vi "Measurement UI.vi"() -> ()   [LabVIEW 2024, in "NIDmmDcRmsMeasurement.lvlib"]
uses:
  NIDmmDCRmsMeasurement.lvlib
panel:
  out "Waveform Data":dbl[](array[numeric]) caption="Waveform Waveform"
  out "Measurement Waveform":waveform(dbl)(graph)
  out "RMS Value":dbl
  out "DC Value":dbl
  out "Signal Out of Range":bool
  in  "Sample Rate (Hz)":dbl=1800000.0 caption="Pin Name" format="%.2p"
  in  "Number of Samples":i32=1000 caption="Sample Rate (Hz)"
  in  "Function":i32(ring)=1003 caption="Measurement Type" items=["Waveform Voltage"=1003, "Waveform Current"=1004]
  in  "Range":dbl=10.0
  in  "Pin Name":string(combo)="Pin1"
  # "Input"
  # "Output"
  # "Pin Settings"
  # "Timing Settings"
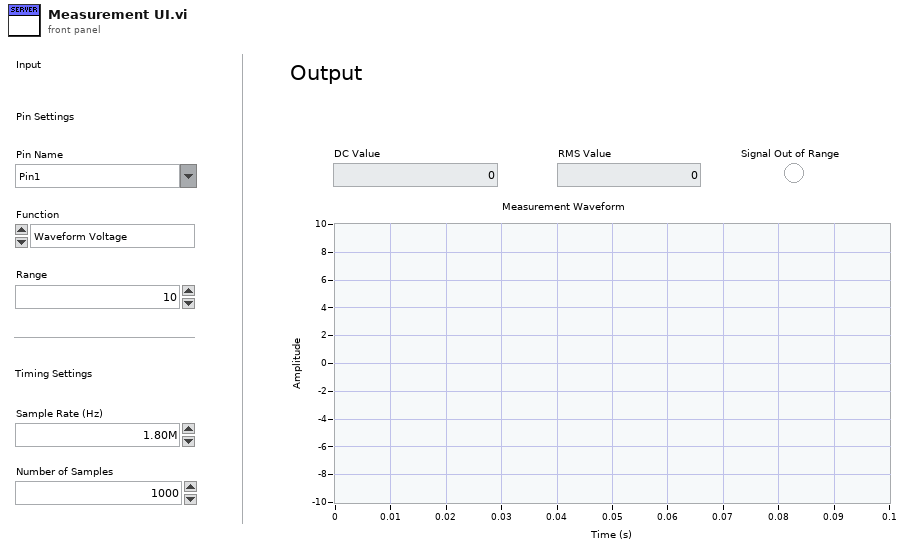
[diagram p1: front panel]
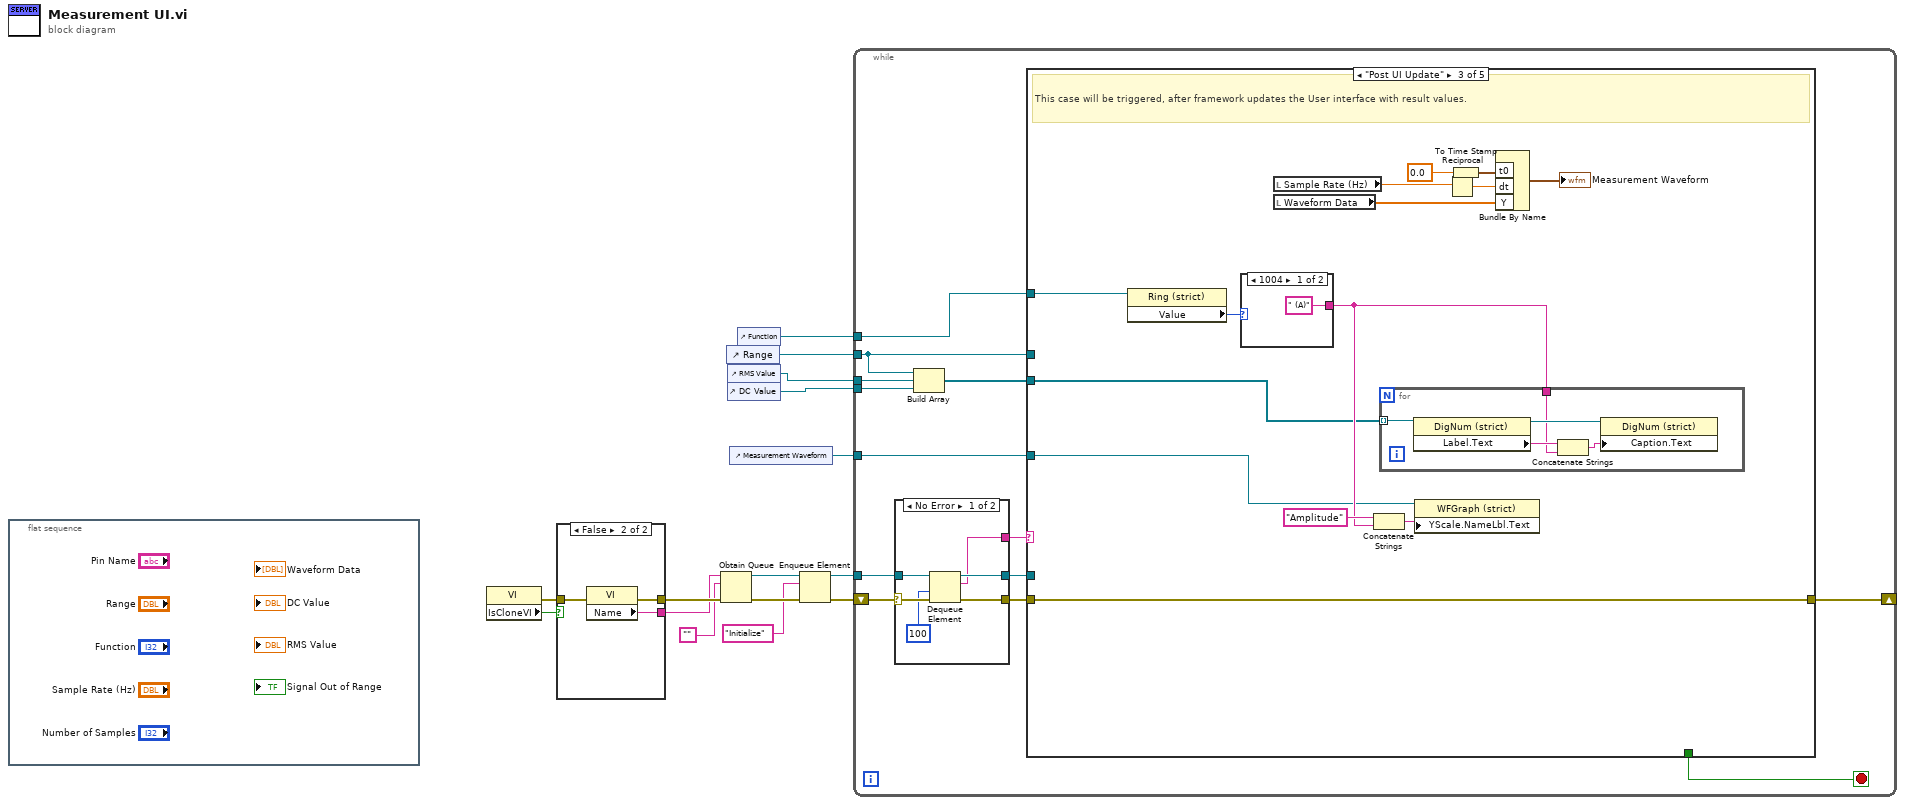
[diagram p0: block diagram]
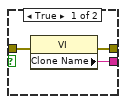
[diagram p2: hidden frame]
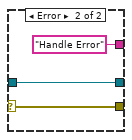
[diagram p3: hidden frame]
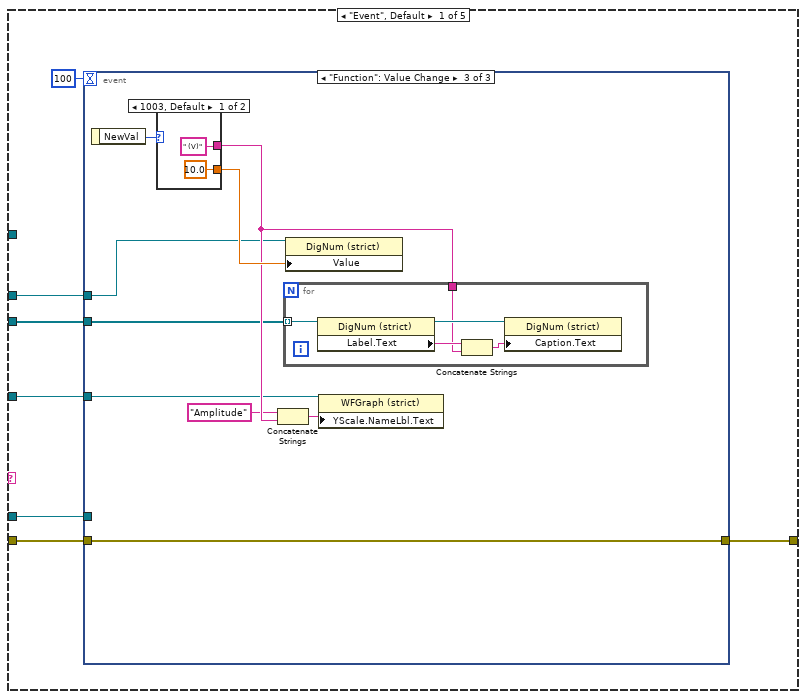
[diagram p4: hidden frame]
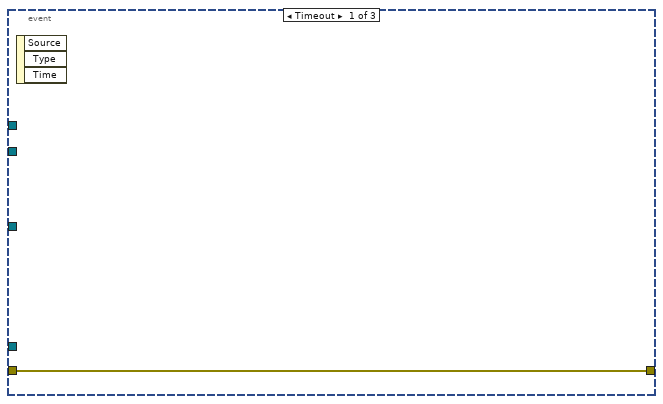
[diagram p5: hidden frame]
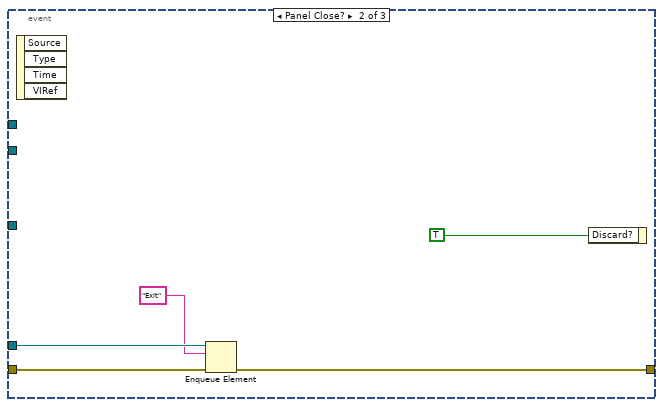
[diagram p6: hidden frame]
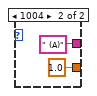
[diagram p7: hidden frame]
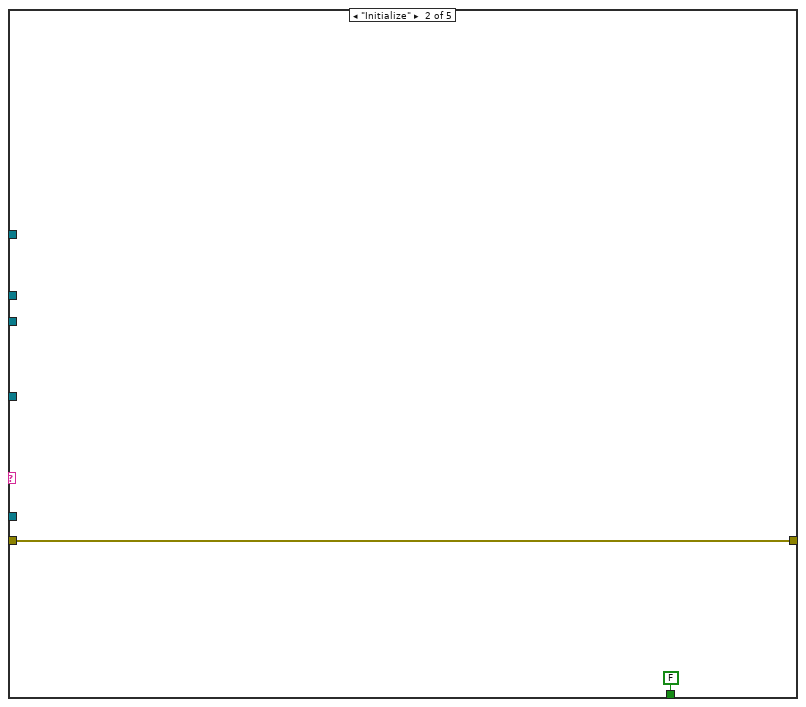
[diagram p8: hidden frame]
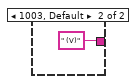
[diagram p9: hidden frame]
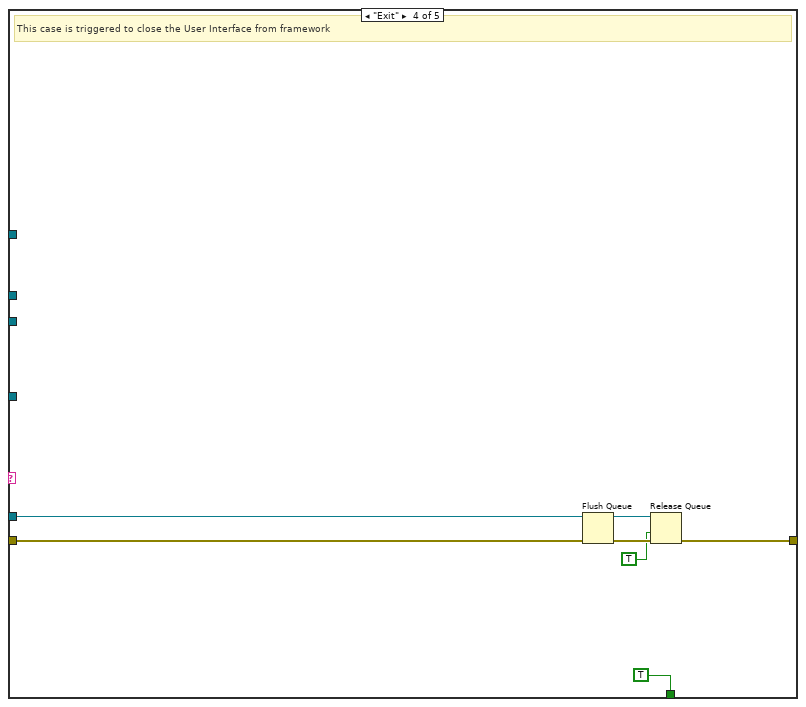
[diagram p10: hidden frame]
diagram:
  n1 = flat-sequence {
    frame #0 {
    }
  }
  n2 = property class="VI"() -> (error out=w6:errorcluster, "IsCloneVI"=w7:bool)  [unwired: 2 in, 1 out]
  n3 = case shown="False" w7 {
    tunnel: [w18 w21] -> w15
    tunnel: [w17 w20] -> w14
    tunnel: w6 -> [w16 w19]
    frame True {
      n4 = property class="VI"(error in=w16) -> (error out=w18:errorcluster, "Clone Name"=w17:string)  [unwired: 1 in, 1 out]
    }
    frame False {
      n5 = property class="VI"(error in=w19) -> (error out=w21:errorcluster, "Name"=w20:string)  [unwired: 1 in, 1 out]
    }
  }
  n6 = Obtain Queue(name (unnamed)=w14, element data type="", error in (no error)=w15) -> (queue out=w11:refnum<queue>, error out=w13:errorcluster)  [unwired: 2 in, 1 out]
  n7 = control-ref of="Range"() -> (w4:refnum<vi>)
  n8 = control-ref of="RMS Value"() -> (w3:refnum<vi>)
  n9 = control-ref of="DC Value"() -> (w2:refnum<vi>)
  n10 = control-ref of="Measurement Waveform"() -> (w5:refnum<vi>)
  n11 = control-ref of="Function"() -> (w1:refnum<vi>)
  n12 = Enqueue Element(queue=w11, element="Initialize", error in (no error)=w13) -> (queue out=w10:refnum<queue>, error out=w12:errorcluster)  [unwired: 1 in, 1 out]
  n13 = while {
    shift-right: [w29] -> _
    shift-left: w12 -> [w34]
    tunnel: w10 -> [w32]
    tunnel: w5 -> [w27]
    tunnel: w4 -> [w26]
    tunnel: w3 -> [w24]
    tunnel: w2 -> [w23]
    tunnel: w1 -> [w25]
    stop <- w28 stop-if-true
    n14 = case shown="No Error" w34 {
      selector: w34 -> [w40 w43]
      tunnel: [w39 w43] -> w33
      tunnel: w32 -> [w38 w42]
      tunnel: [w37 w42] -> w31
      tunnel: [w36 "Handle Error"] -> w30
      frame No Error {
        n15 = Dequeue Element(queue=w38, timeout in ms (-1)=100, error in (no error)=w40) -> (queue out=w37:refnum<queue>, element=w36:string, error out=w39:errorcluster)  [unwired: 1 out]
      }
      frame Error {
      }
    }
    n16 = Build Array(w26, w24, w23) -> (w22:refnum<vi>[])
    n17 = case shown="\"Post UI Update\"" w30 {
      tunnel: w33 -> [w49 w76 w90 w104 w105]
      tunnel: w31 -> [w47 _ _ w102 _]
      tunnel: [w50 w76 w90 w99 w105] -> w29
      tunnel: [_ FALSE _ TRUE _] -> w28
      tunnel: w27 -> [w46 _ w77 _ _]
      tunnel: w26 -> [w45 _ _ _ _]
      tunnel: w25 -> [_ _ w79 _ _]
      tunnel: w22 -> [w44 _ w78 _ _]
      frame "Event", Default {
        n18 = event shown="[2] \"Function\": Value Change" {
          selector: _ -> [_ _ _]
          dyn-events: _ -> [_ _ _]
          timeout: 100 -> [_ _ _]
          tunnel: [w51 w54 w60] -> w50
          tunnel: w49 -> [w51 w55 w60]
          tunnel: w47 -> [_ w53 _]
          tunnel: w46 -> [_ _ w62]
          tunnel: w45 -> [_ _ w61]
          tunnel: w44 -> [_ _ w59]
          event Timeout {
            n19 = event-data() -> ()  [unwired: 1 in, 3 out]
          }
          event Panel Close? {
            n20 = event-data() -> ()  [unwired: 1 in, 4 out]
            n21 = Enqueue Element(queue=w53, element="Exit", error in (no error)=w55) -> (error out=w54:errorcluster)  [unwired: 1 in, 2 out]
            n22 = event-data("Discard?"=TRUE) -> ()  [unwired: 1 in, 1 out]
          }
          event "Function": Value Change {
            n23 = event-data() -> ("NewVal"=w63:i32)  [unwired: 1 in]
            n24 = case shown="1003, Default" w63 {
              tunnel: [" (V)" " (A)"] -> w64
              tunnel: [10.0 ("Value") 1.0 ("Value")] -> w65
              frame 1003, Default {
              }
              frame 1004 {
              }
            }
            n25 = Concatenate Strings("Amplitude", w64) -> (w58:string)
            n26 = for {
              tunnel: w64 -> [w68]
              tunnel: w59 -> [w66] mode=indexing
              n27 = property class="DigNum (strict)"(reference=w66) -> (reference out=w70:refnum<vi>, "Label.Text"=w69:string)  [unwired: 1 in, 1 out]
              n28 = Concatenate Strings(w69, w68) -> (w67:string)
              n29 = property class="DigNum (strict)"(reference=w70, "Caption.Text"=w67) -> ()  [unwired: 1 in, 2 out]
            }
            n30 = property class="DigNum (strict)"(reference=w61, "Value"=w65) -> ()  [unwired: 1 in, 2 out]
            n31 = property class="WFGraph (strict)"(reference=w62, "YScale.NameLbl.Text"=w58) -> ()  [unwired: 1 in, 2 out]
          }
        }
      }
      frame "Initialize" {
      }
      frame "Post UI Update" {
        # "This case will be triggered, after framework updates the User interface with result values."
        n32 = property class="Ring (strict)"(reference=w79) -> ("Value"=w83:i32)  [unwired: 1 in, 2 out]
        n33 = case shown="1004" w83 {
          tunnel: [" (A)" " (V)"] -> w80
          frame 1004 {
          }
          frame 1003, Default {
          }
        }
        n34 = local read "Sample Rate (Hz)"() -> (w86:dbl)
        n35 = local read "Waveform Data"() -> (w85:dbl[])
        n36 = Concatenate Strings("Amplitude", w80) -> (w82:string)
        n37 = for {
          tunnel: w78 -> [w92] mode=indexing
          tunnel: w80 -> [w91]
          n38 = property class="DigNum (strict)"(reference=w92) -> (reference out=w95:refnum<vi>, "Label.Text"=w94:string)  [unwired: 1 in, 1 out]
          n39 = Concatenate Strings(w94, w91) -> (w93:string)
          n40 = property class="DigNum (strict)"(reference=w95, "Caption.Text"=w93) -> ()  [unwired: 1 in, 2 out]
        }
        n41 = property class="WFGraph (strict)"(reference=w77, "YScale.NameLbl.Text"=w82) -> ()  [unwired: 1 in, 2 out]
        n42 = Reciprocal(x=w86) -> (1/x=w89:dbl)
        n43 = To Time Stamp(1:0.0 ("t0")) -> (0:w87:timestamp)
        n44 = Bundle By Name("t0"=w87, "dt"=w89, "Y"=w85) -> (→"Measurement Waveform":waveform(dbl))  [unwired: 1 in]
      }
      frame "Exit" {
        # "This case is triggered to close the User Interface from framework"
        n45 = Flush Queue(queue=w102, error in (no error)=w104) -> (queue out=w101:refnum<queue>, error out=w100:errorcluster)  [unwired: 1 out]
        n46 = Release Queue(queue=w101, force destroy? (F)=TRUE, error in (no error)=w100) -> (error out=w99:errorcluster)  [unwired: 2 out]
      }
      frame "Handle Error" {
      }
    }
  }
